vi "Test Process within App Log Error Message When Setting Handler After Process.vi"(8 "error in (no error)":errorcluster, 11 "Test Case In":refnum<class "Logger Test.lvclass">) -> (0 "error out":errorcluster, 3 "Test Case Out":refnum<class "Logger Test.lvclass">)   [LabVIEW 2020, in "Logger Test.lvclass"]
uses:
  Logger Test.lvclass
  C:/Program Files (x86)/National Instruments/LabVIEW 2020/vi.lib/Astemes/LUnit/Test Case.lvclass
  source/Framework Test Suite/Mock Process/Mock Process.lvclass
  C:/git/astemes-triarc-framework/source/Framework/Process/Process.lvclass
  C:/git/astemes-triarc-framework/source/Framework/Logging/Logging.lvclass
  source/Framework/Application/Application.lvclass
  source/Framework Test Suite/Mock Log Handler/Mock Log Handler.lvclass
  source/Framework/Process/Process.lvclass/Process.ctl
  source/Framework/Application/Application.lvclass/Application.ctl
  <vilib>/Astemes/LUnit/Test Case.lvclass/Test Case.ctl
  07009c05-29cc-44a3-a854-ccf813a5e6df.vi
  6e911bec-e8a5-4451-b4a0-22b7fdbbda38.vi
  34049daa-a343-404c-9e84-4ab9e23fdc36.vi
  source/Framework/Application/Private/Add Process to Map.vi
  source/Framework/Application/Private/Throw Error If Process Already in App.vi
  source/Framework/Process/Protected/Messaging/Send Message.vi
  source/Framework/Process/Public/Lifecycle/Get Lifecycle State.vi
  source/Framework/Process/Protected/SubVIs/Set Context.vi
  source/Framework/Process/Private/SubVIs/Wait for finish.vi
  source/Framework/Process/Private/SubVIs/Set Lifecycle State.vi
  source/Framework/Application/Private/Retrieve Process from App.vi
  source/Framework/Application/Private/Parse Process Name.vi
  source/Framework/Application/Private/Get Process from Map.vi
  <vilib>/Astemes/LUnit/Append Pass Result.vi
  <vilib>/Astemes/LUnit/Append Fail Result.vi
  <vilib>/Astemes/LUnit/Describe Comparison.vi
  <vilib>/Astemes/LUnit/Compare Variants.vi
  source/Framework/Process/Private/SubVIs/Handle Debug Data.vi
  source/Framework/Process/Protected/Messaging/Request Message.vi
  <vilib>/AdvancedString/Delimited String to 1D String Array.vi
  <vilib>/Astemes/LUnit/Variant to string.vi
  source/Framework/Logging/Log Debug.vi
  <vilib>/AdvancedString/1D String Array to Delimited String.vi
  <vilib>/Utility/High Resolution Relative Seconds.vi
  source/Framework/Process/Private/SubVIs/Enqueue Request Message.vi
  source/Framework/Process/Process.lvclass
  <vilib>/Utility/error.llb/Error Cluster From Error Code.vi
  source/Framework/Process/Public/Read Name.vi
  source/Framework/Process/Private/SubVIs/Wait for Response Message.vi
  <vilib>/Utility/Data Type/Get Type Information.vi
  <vilib>/Utility/LVClass/Get LV Class Name.vi
  source/Framework/Logging/Logging.lvclass
  source/Framework Test Suite/Support/Test Support.lvlib
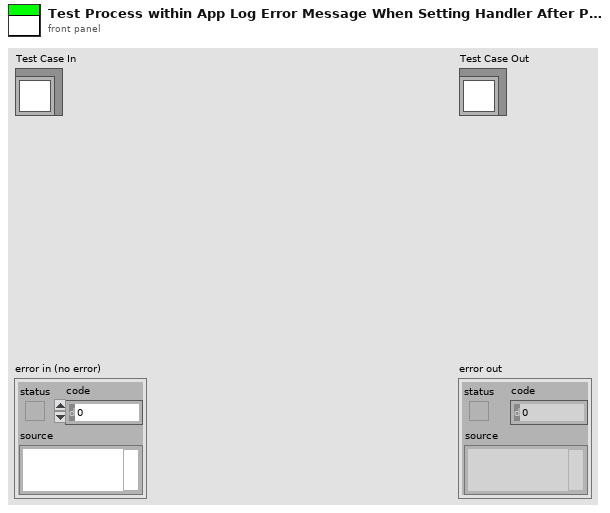
[diagram p1: front panel]
types:
  T1 = typedef "Mock Log Handler.lvclass/Log Entry.ctl" = cluster{"Level":string, "Source":string, "Message":string}
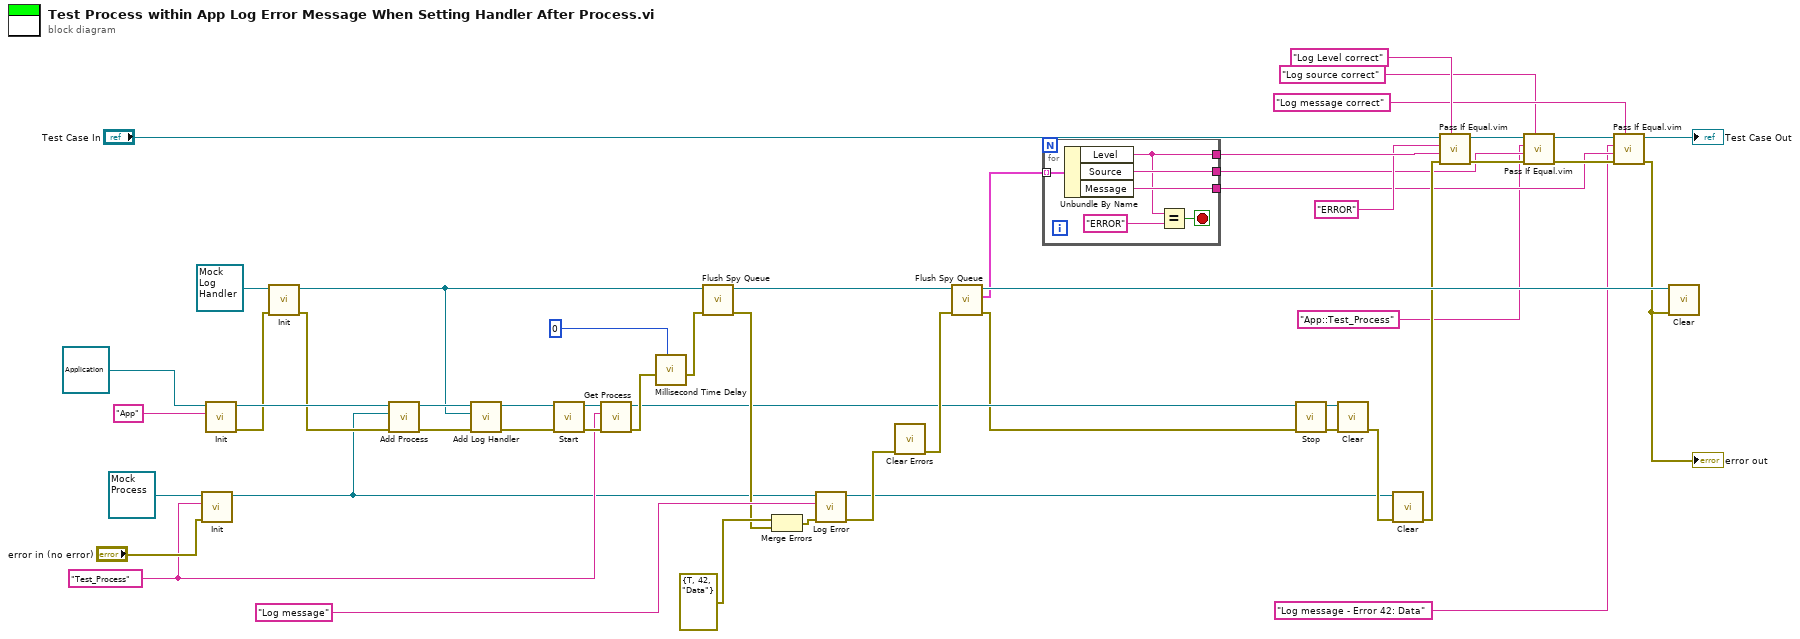
[diagram p0: block diagram]
diagram:
  w5 = "Test_Process" ("Name")
  n1 = call-dynamic "Init.vi"("error in (no error)"="error in (no error)", "Name"=w5, "Mock Process In"=refnum<class "Mock Process.lvclass"> refnum) -> ("Mock Process Out"=w4:refnum<class "Mock Process.lvclass">)  [unwired: 7 in, 1 out]
  n2 = call-dynamic "Init.vi"("Name"="App", "Process In"=refnum<class "Application.lvclass"> refnum ("Application.lvclass")) -> ("error out"=w46:errorcluster, "Process Out"=w49:refnum<class "Application.lvclass">)  [unwired: 8 in]
  n3 = call-dynamic "Init.vi"("error in (no error)"=w46, "Mock Log Handler In"=refnum<class "Mock Log Handler.lvclass"> refnum ("Mock Log Handler.lvclass")) -> ("error out"=w45:errorcluster, "Mock Log Handler Out"=w9:refnum<class "Mock Log Handler.lvclass">)  [unwired: 8 in]
  n4 = call "Add Process.vi"("error in (no error)"=w45, "Process"=w4, "Application In"=w49) -> ("error out"=w22:errorcluster, "Application Out"=w11:refnum<class "Application.lvclass">)  [unwired: 7 in]
  n5 = call "Add Log Handler.vi"("error in (no error)"=w22, "Log Handler"=w9, "Process In"=w11) -> ("error out"=w12:errorcluster, "Process Out"=w10:refnum<class "Application.lvclass">)  [unwired: 7 in]
  n6 = call "Start.vi"("error in (no error)"=w12, "Process In"=w10) -> ("error out"=w16:errorcluster, "Process Out"=w7:refnum<class "Application.lvclass">)  [unwired: 7 in, 1 out]
  n7 = call "Get Process.vi"("error in (no error)"=w16, "Process Name"=w5, "Application In"=w7) -> ("error out"=w8:errorcluster, "Application Out"=w6:refnum<class "Application.lvclass">)  [unwired: 6 in, 1 out]
  n8 = call "Millisecond Time Delay.vi"("milliseconds to wait"=u32 0, "error in (no error)"=w8) -> ("error out"=w14:errorcluster)  [unwired: 7 in]
  n9 = call "Flush Spy Queue.vi"("error in (no error)"=w14, "Mock Log Handler in"=w9) -> ("error out"=w15:errorcluster, "Mock Log Handler out"=w17:refnum<class "Mock Log Handler.lvclass">)  [unwired: 7 in, 1 out]
  n10 = Merge Errors(errorcluster {"status"=TRUE, "code"=42, "source"="Data"} ("error in (no error)"), w15) -> (w19:errorcluster)
  n11 = call "Log Error.vi"("error in (no error)"=w19, "Message"="Log message", "Logging In"=w4) -> ("error out"=w29:errorcluster, "Logging Out"=w3:refnum<class "Mock Process.lvclass">)  [unwired: 7 in]
  n12 = call <vilib>:"Clear Errors.vi"("error in (no error)"=w29) -> ("error out"=w28:errorcluster)  [unwired: 5 in, 1 out]
  n13 = call "Flush Spy Queue.vi"("error in (no error)"=w28, "Mock Log Handler in"=w17) -> ("error out"=w2:errorcluster, "remaining elements"=w43:T1[], "Mock Log Handler out"=w44:refnum<class "Mock Log Handler.lvclass">)  [unwired: 7 in]
  n14 = for {
    tunnel: w43 -> [w58] mode=indexing
    tunnel: [w54] -> w42
    tunnel: [w57] -> w33
    tunnel: [w56] -> w32
    stop <- w53 stop-if-true
    n15 = Unbundle By Name(w58) -> ("Level"=w54:string, "Source"=w57:string, "Message"=w56:string)
    n16 = Equal?(x=w54, y="ERROR") -> (x = y?=w53:bool)
  }
  n17 = call "Stop.vi"("error in (no error)"=w2, "Process In"=w6) -> ("error out"=w21:errorcluster, "Process Out"=w20:refnum<class "Application.lvclass">)  [unwired: 7 in, 1 out]
  n18 = call-dynamic "Clear.vi"("error in (no error)"=w21, "Application In"=w20) -> ("error out"=w48:errorcluster)  [unwired: 9 in]
  n19 = call-dynamic "Clear.vi"("error in (no error)"=w48, "Mock Process In"=w3) -> ("error out"=w36:errorcluster)  [unwired: 9 in]
  n20 = call "Pass If Equal.vim"("Description"="Log Level correct", "error in (no error)"=w36, "Actual"=w42, "Expected"="ERROR", "LUnit Test Case In"="Test Case In") -> ("error out"=w38:errorcluster, "LUnit Test Case Out"=w51:refnum<class "Logger Test.lvclass">)  [unwired: 5 in]
  n21 = call "Pass If Equal.vim"("Description"="Log source correct", "error in (no error)"=w38, "Actual"=w33, "Expected"="App::Test_Process" ("Name"), "LUnit Test Case In"=w51) -> ("error out"=w37:errorcluster, "LUnit Test Case Out"=w40:refnum<class "Logger Test.lvclass">)  [unwired: 5 in]
  n22 = call "Pass If Equal.vim"("Description"="Log message correct", "error in (no error)"=w37, "Actual"=w32, "Expected"="Log message - Error 42: Data" ("Message"), "LUnit Test Case In"=w40) -> ("error out"=w1:errorcluster, "LUnit Test Case Out"=→"Test Case Out":refnum<class "Logger Test.lvclass">)  [unwired: 5 in]
  "error out" <- w1
  n23 = call-dynamic "Clear.vi"("error in (no error)"=w1, "Mock Log Handler In"=w44) -> ()  [unwired: 9 in, 1 out]
